vi "AO Python Interface.vi"(7 "Calling VI Ref":refnum<vi>) -> ()   [LabVIEW 2016]
uses:
  AO Python Controls/AO Python Data Type.ctl
  AO Python Controls/AO Python Units.ctl
  AO Python Controls/AO Python Vector Type.ctl
  AO Python Controls/AO Python Update Type.ctl
  AO Python Controls/AO Python Notifier Element.ctl
  AO Python Controls/AO Python Actions.ctl
  Hardware Configuration/Hardware Configuration Controls/Device Type.ctl
  Hardware Configuration/Hardware Configuration Controls/Device Function.ctl
  AO Python Controls/AO Python System Configuration.ctl
  AO Python Controls/AO Python Command List Type.ctl
  AO Python Controls/AO Python Next Command Type.ctl
  AO Python Controls/AO Python Image Type.ctl
  AO Python Controls/AO Python Status Type.ctl
panel:
  out "Current Image":u16[][](graph)
  in  "Use ROI":bool
  out "Python Status":string
  out "Command List":string[](array[string])
  in  "Fake Image":bool
  out "Command from Python":string
  in  "AO Data":T1={"LVCommand"="run_sensorless", "vector"=[], "flat_on"=1, "units"=enum."rad", "vector_type"=enum."zernike", "update_type"=enum."absolute"}
  in  "Send Command":bool
  in  "Quit":bool
  # "run_sensorless\nupdate\nquery_commands"
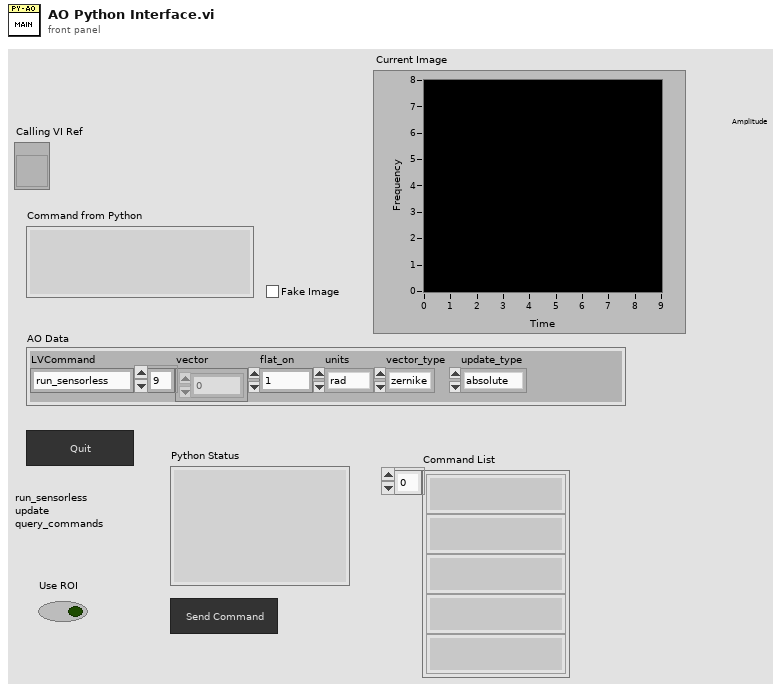
[diagram p1: front panel]
types:
  T1 = typedef "AO Python Data Type.ctl" = cluster{"LVCommand":string, "vector":dbl[], "flat_on":i32, "units":T2, "vector_type":T3, "update_type":T4}
  T2 = typedef "AO Python Units.ctl" = enum16{"rad", "nm"}
  T3 = typedef "AO Python Vector Type.ctl" = enum16{"zernike", "actuators", "zernike_highNA", "dm_modes1"}
  T4 = typedef "AO Python Update Type.ctl" = enum16{"absolute", "relative"}
  T5 = typedef "AO Python Actions.ctl" = enum16{"Error Check", "Open Connection", "Send Configuration", "Send Command", "Wait for Command", "Get Image", "Update DM", "Get Status", "Quit"}
  T6 = typedef "AO Python Notifier Element.ctl" = cluster{"Actions":T5, "Received?":bool, "Running?":bool, "AO Data":T1, "Command List":string[], "Python Status":string, "Error":errorcluster}
  T7 = typedef "Device Function.ctl" = enum16{"Primary", "Secondary", "Overview", "Wide Field Drift Correction", "642 nm Excitation", "560 nm Excitation", "546 nm Excitation", "488 nm Excitation", "405 nm Excitation", "Objective Drift Correction", "Objective XY", "Objective Z", "Sample XY", "Sample Coarse Z", "Sample Z", "4Pi Lower", "4Pi Upper", "Adj Cavity"}
  T8 = typedef "Device Type.ctl" = enum16{"AOTF", "Camera", "Deformable Mirror", "Laser", "Shutter", "Stage"}
  T9 = typedef "AO Python Command List Type.ctl" = cluster{"CommandList":string[]}
  T10 = typedef "AO Python System Configuration.ctl" = cluster{"stack_size":u16[], "fov":dbl[]}
  T11 = typedef "AO Python Next Command Type.ctl" = cluster{"NextCommand":string}
  T12 = typedef "AO Python Image Type.ctl" = cluster{"stack":dbl[][][]}
  T13 = typedef "AO Python Status Type.ctl" = cluster{"ack":string}
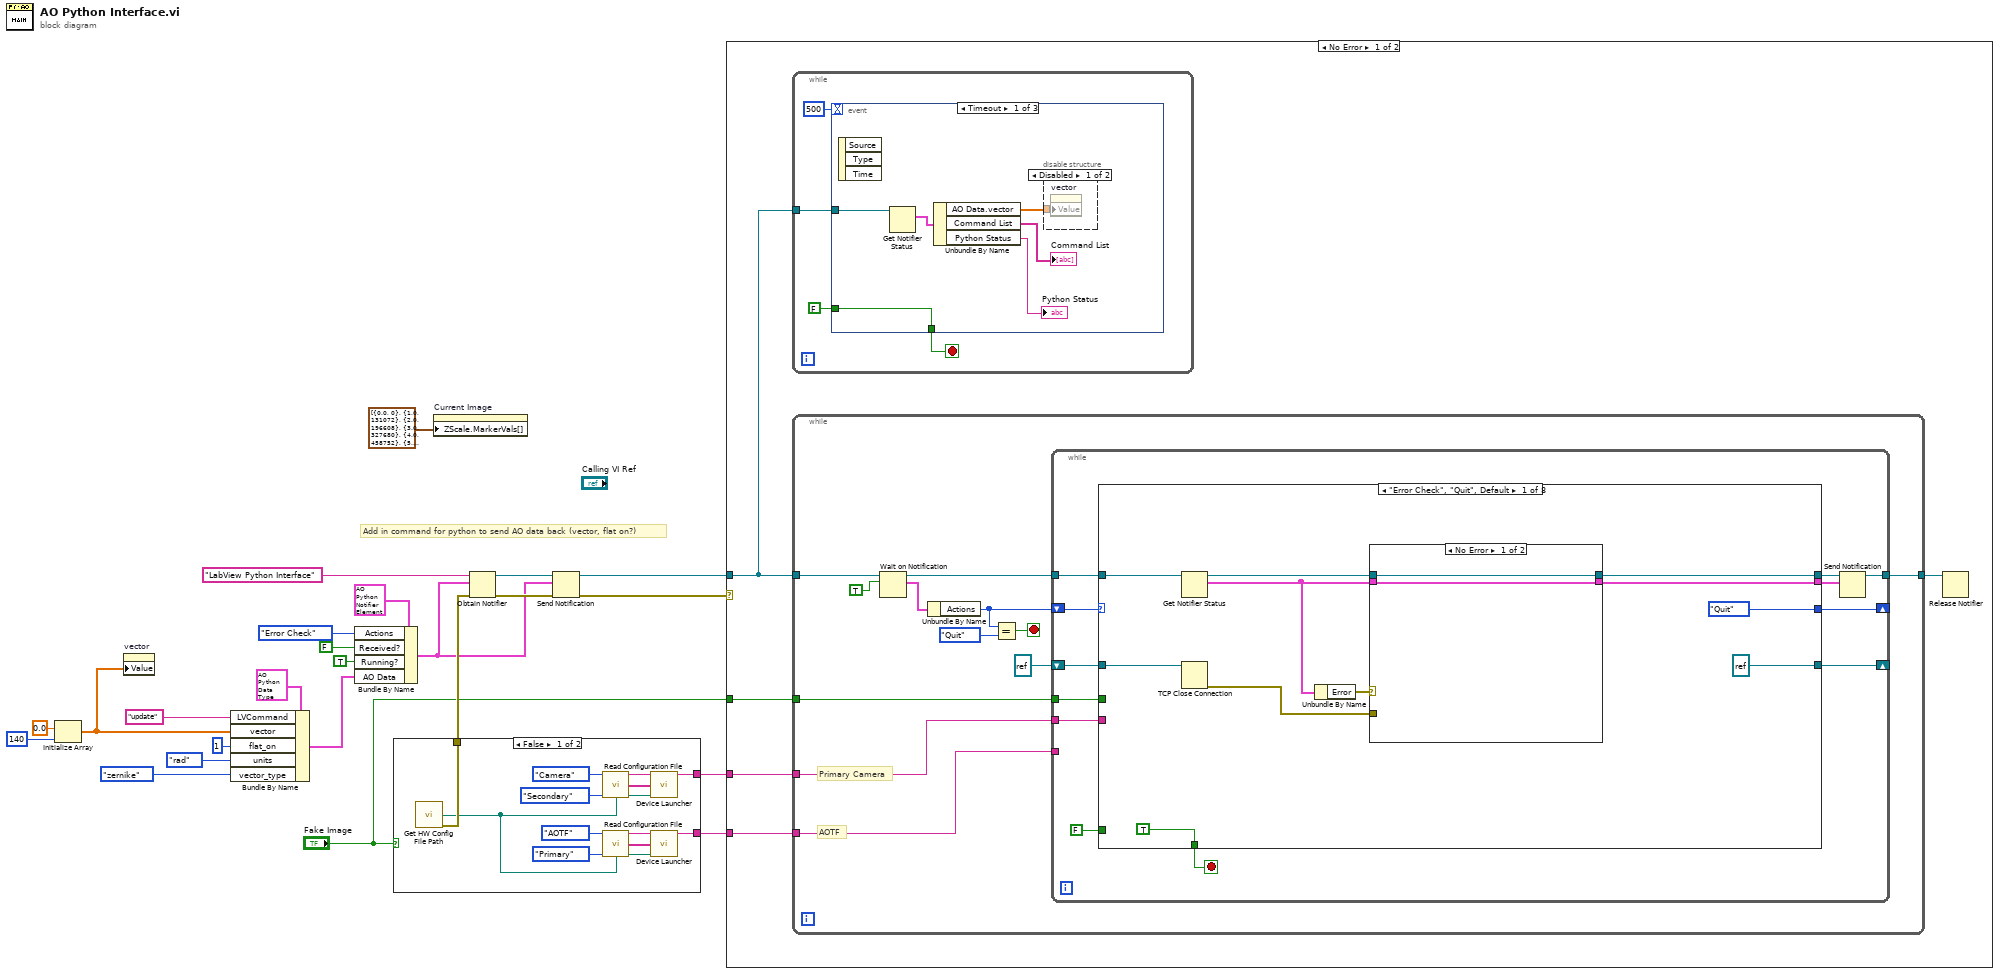
[diagram p0: block diagram]
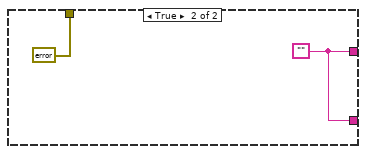
[diagram p2: hidden frame]
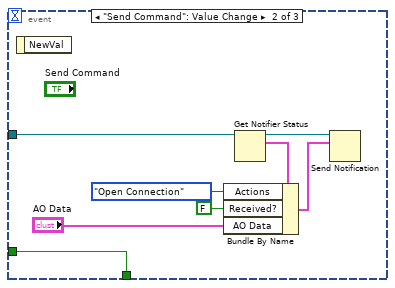
[diagram p4: hidden frame]
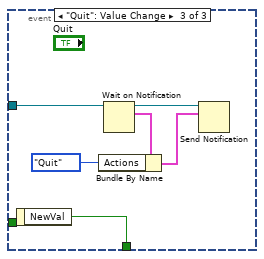
[diagram p5: hidden frame]
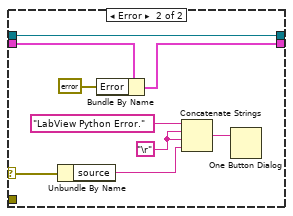
[diagram p6: hidden frame]
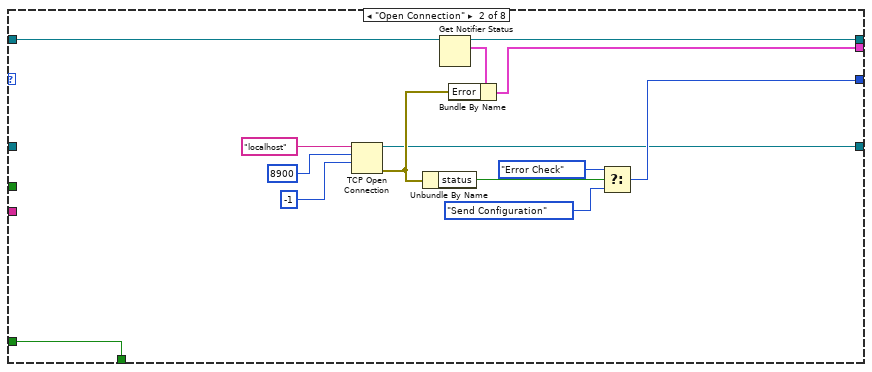
[diagram p7: hidden frame]
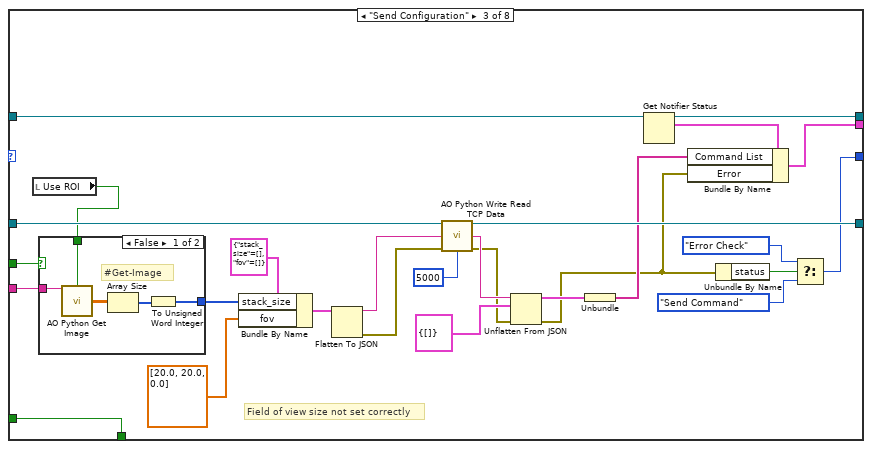
[diagram p8: hidden frame]
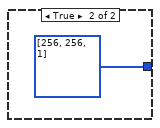
[diagram p9: hidden frame]
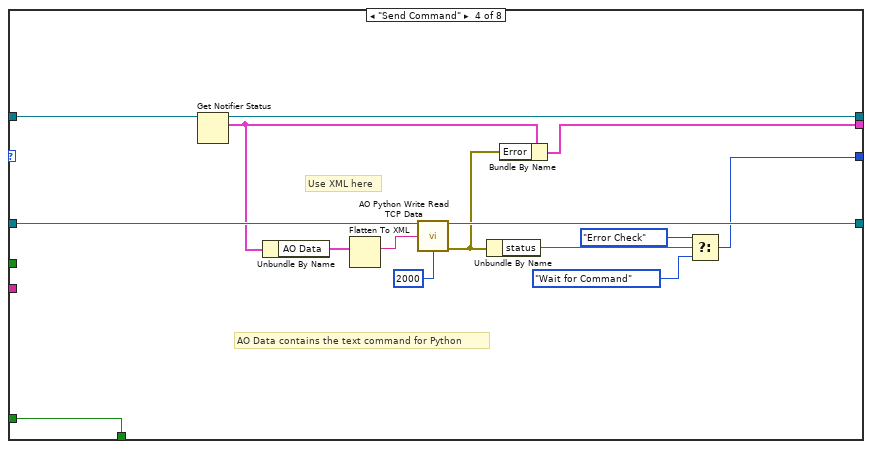
[diagram p10: hidden frame]
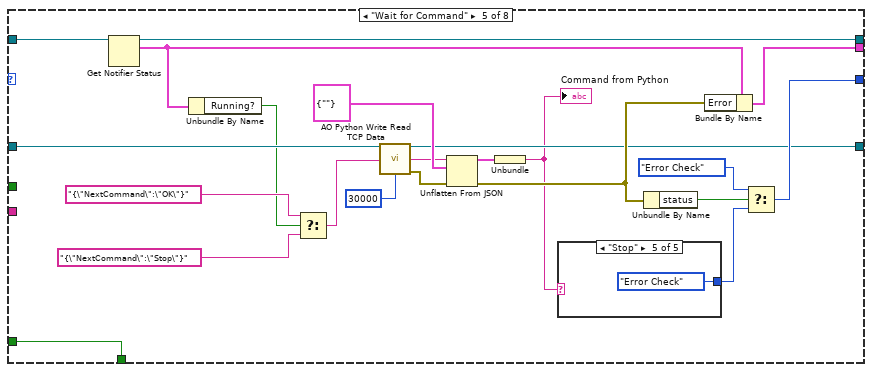
[diagram p11: hidden frame]
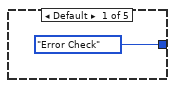
[diagram p12: hidden frame]
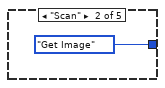
[diagram p13: hidden frame]
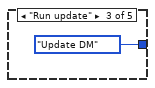
[diagram p14: hidden frame]
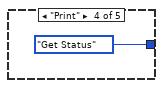
[diagram p15: hidden frame]
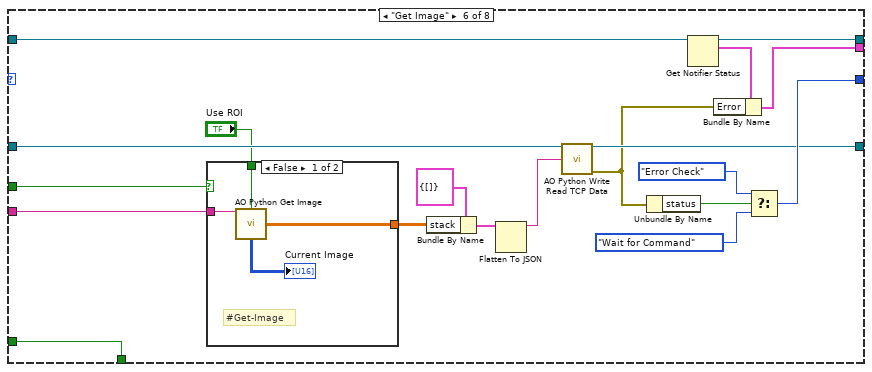
[diagram p16: hidden frame]
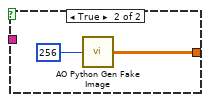
[diagram p17: hidden frame]
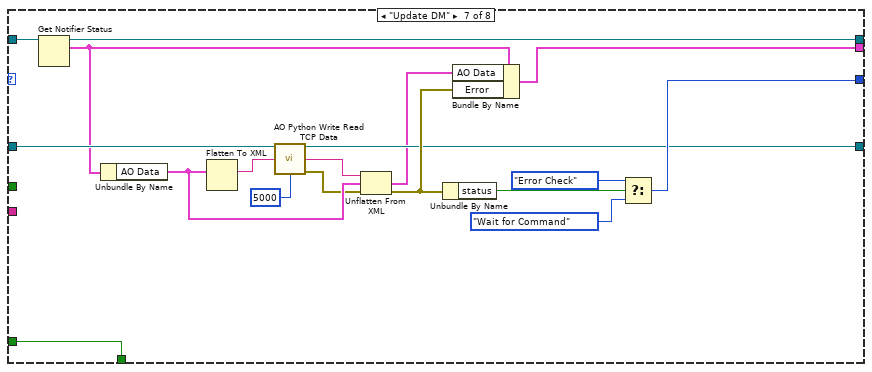
[diagram p18: hidden frame]
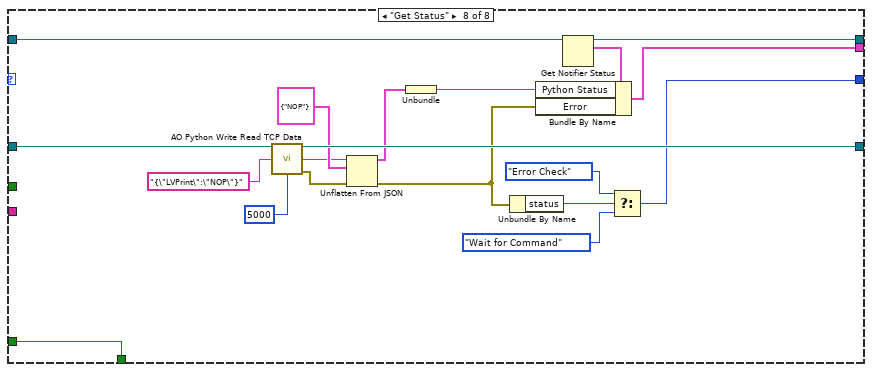
[diagram p19: hidden frame]
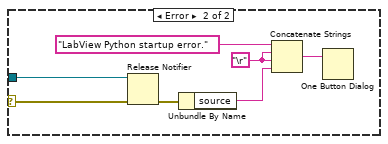
[diagram p20: hidden frame]
diagram:
  # "Add in command for python to send AO data back (vector, flat on?)"
  n1 = Initialize Array(0.0 ("element"), 140 ("dimension size")) -> (w1:dbl[])
  n2 = property on="vector" class="Arr (strict)"("Value"=w1) -> ()  [unwired: 2 in, 2 out]
  n3 = Bundle By Name(cluster=T1 {"LVCommand"="Default", "vector"=[], "flat_on"=1, "units"=enum."rad", "vector_type"=enum."zernike", "update_type"=enum."absolute"} ("input cluster"), "LVCommand"="update", "vector"=w1, "flat_on"=1 ("Flat On?"), "units"=AO_Python_Units."rad" ("Units"), "vector_type"=AO_Python_Vector_Type."zernike" ("Vector Type")) -> (w10:T1)
  n4 = Bundle By Name(cluster=T6 {"Actions"=enum."Send Command", "Received?"=FALSE, "Running?"=FALSE, "AO Data"={"LVCommand"="", "vector"=[], "flat_on"=1, "units"=enum."rad", "vector_type"=enum."zernike", "update_type"=enum."absolute"}, "Command List"=[], "Python Status"="", "Error"={"status"=FALSE, "code"=0, "source"=""}} ("LabView Python Notifier Element"), "Actions"=AO_Python_Actions."Error Check", "Received?"=FALSE, "Running?"=TRUE, "AO Data"=w10) -> (w4:T6)
  n5 = case shown="False" "Fake Image" {
    tunnel: [w38 w39] -> w23
    tunnel: [w37 errorcluster {"status"=FALSE, "code"=0, "source"=""} ("Error")] -> w22
    tunnel: [w35 w39] -> w21
    frame False {
      n6 = call "Get HW Config File Path.vi"() -> ("File Path"=w36:path, "Error"=w37:errorcluster)  [unwired: 14 in]
      n7 = call "Read Configuration File.vi"("Device Type"=Device_Type."Camera", "Device Function"=Device_Function."Secondary", "Config File Path"=w36) -> ("Unique Notifier Name"=w34:string, "Device Ports/IDs/Channels"=w33:string[], "Device Engine Path"=w32:path)  [unwired: 9 in, 1 out]
      n8 = call "Read Configuration File.vi"("Device Type"=Device_Type."AOTF", "Device Function"=Device_Function."Primary", "Config File Path"=w36) -> ("Unique Notifier Name"=w25:string, "Device Ports/IDs/Channels"=w26:string[], "Device Engine Path"=w27:path)  [unwired: 9 in, 1 out]
      n9 = call "Device Launcher.vi"("Notifier Name"=w34, "Device Ports/IDs/Channels"=w33, "Device Engine Path"=w32) -> ("Notifier Name"=w38:string)  [unwired: 11 in, 1 out]
      n10 = call "Device Launcher.vi"("Notifier Name"=w25, "Device Ports/IDs/Channels"=w26, "Device Engine Path"=w27) -> ("Notifier Name"=w35:string)  [unwired: 11 in, 1 out]
    }
    frame True {
      w39 = ""
    }
  }
  n11 = property on="Current Image" class="IntGraph (strict)"("ZScale.MarkerVals[]"=cluster{dbl, u32}[] [{0.0, 0}, {1.0, 131072}, {2.0, 196608}, {3.0, 327680}, {4.0, 458752}, {5.0, 589824}, {6.0, 720896}, {7.0, 851971}, {8.0, 983043}, {9.0, 1114115}, {10.0, 1245187}, {11.0, 1376259}, {12.0, 1507331}, {13.0, 1638403}, {14.0, 1769475}, {15.0, 1769479}, {16.0, 2031623}, {17.0, 2162695}, {18.0, 2293767}, {19.0, 2424839}, {20.0, 2555911}, {21.0, 2686983}, {22.0, 2818055}, {23.0, 2949127}, {24.0, 3080203}, {25.0, 3211275}, {26.0, 3342347}, {27.0, 3473419}, {28.0, 3604491}, {29.0, 3735563}, {30.0, 3866635}, {31.0, 3867403}, {32.0, 4129547}, {33.0, 4260619}, {34.0, 4391691}, {35.0, 4522763}, {36.0, 4653839}, {37.0, 4784911}, {38.0, 4915983}, {39.0, 5178127}, {40.0, 5309199}, {41.0, 5440271}, {42.0, 5571343}, {43.0, 5702415}, {44.0, 5703439}, {45.0, 5965583}, {46.0, 6096655}, {47.0, 6227727}, {48.0, 6358799}, {49.0, 6489871}, {50.0, 6620943}, {51.0, 6752015}, {52.0, 6883087}, {53.0, 7015183}, {54.0, 7146255}, {55.0, 7277327}, {56.0, 7408399}, {57.0, 7539471}, {58.0, 7670543}, {59.0, 7801615}, {60.0, 8063759}, {61.0, 8194831}, {62.0, 8326927}, {63.0, 8457999}, {64.0, 8589075}, {65.0, 8720147}, {66.0, 8851219}, {67.0, 8982291}, {68.0, 9113363}, {69.0, 9114387}, {70.0, 9376531}, {71.0, 9507603}, {72.0, 9638675}, {73.0, 9769747}, {74.0, 9901843}, {75.0, 10032915}, {76.0, 10163987}, {77.0, 10229523}, {78.0, 10295059}, {79.0, 10427155}, {80.0, 10558227}, {81.0, 10689299}, {82.0, 10820371}, {83.0, 10886931}, {84.0, 10952467}, {85.0, 11083539}, {86.0, 11214611}, {87.0, 11215635}, {88.0, 11477779}, {89.0, 11543315}, {90.0, 11608851}, {91.0, 11740947}, {92.0, 11806483}, {93.0, 11872019}, {94.0, 12004115}, {95.0, 12135187}, {96.0, 12266259}, {97.0, 12267283}, {98.0, 12398355}, {99.0, 12529427}, {100.0, 12530451}, {101.0, 12595987}, {102.0, 12530451}, {103.0, 12793619}, {104.0, 12794131}, {105.0, 12794643}, {106.0, 13056787}, {107.0, 13057299}, {108.0, 13057811}, {109.0, 13188883}, {110.0, 13320979}, {111.0, 13386515}, {112.0, 13452563}, {113.0, 13584147}, {114.0, 13584659}, {115.0, 13585171}, {116.0, 13585683}, {117.0, 13717267}, {118.0, 13848339}, {119.0, 13849363}, {120.0, 13849875}, {121.0, 13850387}, {122.0, 13981459}, {123.0, 14113555}, {124.0, 14114067}, {125.0, 14114579}, {126.0, 14115091}, {127.0, 14246675}, {128.0, 14377747}, {129.0, 14378771}, {130.0, 14379283}, {131.0, 14379539}, {132.0, 14379795}, {133.0, 14380819}, {134.0, 14511891}, {135.0, 14643987}, {136.0, 14644503}, {137.0, 14645015}, {138.0, 14645527}, {139.0, 14646039}, {140.0, 14646551}, {141.0, 14778135}, {142.0, 14909207}, {143.0, 14910231}, {144.0, 14910747}, {145.0, 14911259}, {146.0, 14911771}, {147.0, 14912283}, {148.0, 14912797}, {149.0, 15044383}, {150.0, 15175455}, {151.0, 15175967}, {152.0, 15176479}, {153.0, 15176991}, {154.0, 15177507}, {155.0, 15178019}, {156.0, 15178531}, {157.0, 15310115}, {158.0, 15441701}, {159.0, 15441959}, {160.0, 15442215}, {161.0, 15442727}, {162.0, 15443243}, {163.0, 15443755}, {164.0, 15444269}, {165.0, 15444783}, {166.0, 15444783}, {167.0, 15576367}, {168.0, 15707953}, {169.0, 15708467}, {170.0, 15708979}, {171.0, 15708981}, {172.0, 15708983}, {173.0, 15710011}, {174.0, 15710523}, {175.0, 15711037}, {176.0, 15711039}, {177.0, 15711553}, {178.0, 15843139}, {179.0, 15974213}, {180.0, 15974215}, {181.0, 15974217}, {182.0, 15974219}, {183.0, 15975755}, {184.0, 15976271}, {185.0, 15976785}, {186.0, 15977299}, {187.0, 15977301}, {188.0, 15977815}, {189.0, 15978327}, {190.0, 15978331}, {191.0, 16109917}, {192.0, 16241503}, {193.0, 16241505}, {194.0, 16242019}, {195.0, 16242535}, {196.0, 16242537}, {197.0, 16242539}, {198.0, 16243563}, {199.0, 16243567}, {200.0, 16244081}, {201.0, 16244595}, {202.0, 16244599}, {203.0, 16244601}, {204.0, 16244603}, {205.0, 16245627}, {206.0, 16245631}, {207.0, 16245633}, {208.0, 16246147}, {209.0, 16246663}, {210.0, 16377735}, {211.0, 16508811}, {212.0, 16508815}, {213.0, 16509839}, {214.0, 16509843}, {215.0, 16509845}, {216.0, 16509847}, {217.0, 16510361}, {218.0, 16510875}, {219.0, 16510879}, {220.0, 16510881}, {221.0, 16510883}, {222.0, 16511399}, {223.0, 16511911}, {224.0, 16511915}, {225.0, 16511917}, {226.0, 16511919}, {227.0, 16511923}, {228.0, 16512437}, {229.0, 16512951}, {230.0, 16512955}, {231.0, 16512957}, {232.0, 16512959}, {233.0, 16512961}, {234.0, 16512963}, {235.0, 16512967}, {236.0, 16513481}, {237.0, 16513995}, {238.0, 16513999}, {239.0, 16514001}, {240.0, 16514003}, {241.0, 16514005}, {242.0, 16514007}, {243.0, 16514011}, {244.0, 16514013}, {245.0, 16514015}, {246.0, 16514019}, {247.0, 16514021}, {248.0, 16514023}, {249.0, 16514027}, {250.0, 16514029}, {251.0, 16514031}, {252.0, 16514035}, {253.0, 16514037}, {254.0, 16514039}, {255.0, 16514043}] ("Z Scale.Marker Values[]")) -> ()  [unwired: 2 in, 2 out]
  n12 = Obtain Notifier(name (unnamed)="LabView Python Interface", notification data type=w4, error in (no error)=w22) -> (notifier out=w8:refnum<notifier>, error out=w7:errorcluster)  [unwired: 1 in, 1 out]
  n13 = Send Notification(notification=w4, notifier=w8, error in (no error)=w7) -> (notifier out=w6:refnum<notifier>, error out=w5:errorcluster)
  n14 = case shown="No Error" w5 {
    selector: w5 -> [_ w268]
    tunnel: w6 -> [w42 w274]
    tunnel: w23 -> [w45 _]
    tunnel: w21 -> [w43 _]
    tunnel: "Fake Image" -> [w41 _]
    frame No Error {
      n15 = while {
        tunnel: w42 -> [w47]
        stop <- w49 stop-if-true
        n16 = event shown="[0] Timeout" {
          selector: _ -> [_ _ _]
          dyn-events: _ -> [_ _ _]
          timeout: 500 -> [_ _ _]
          tunnel: [w55 w64 w70] -> w49
          tunnel: FALSE -> [w55 w64 _]
          tunnel: w47 -> [w54 w59 w69]
          event Timeout {
            n17 = event-data() -> ()  [unwired: 1 in, 3 out]
            n18 = Get Notifier Status(notifier=w54) -> (current notification=w53:T6)  [unwired: 1 in, 4 out]
            n19 = Unbundle By Name(w53) -> ("AO Data.vector"=w52:dbl[], "Command List"=→"Command List":string[], "Python Status"=→"Python Status":string)
            n20 = disable-structure shown="Disabled" {
              disable-tunnel: w52 -> [w56 _]
              frame Disabled {
                n21 = property on="vector" class="Arr (strict)"("Value"=w56) -> ()  [unwired: 2 in, 2 out]
              }
              frame Enabled {
              }
            }
          }
          event "Send Command": Value Change {
            n22 = event-data() -> ()  [unwired: 1 in, 1 out]
            n23 = Get Notifier Status(notifier=w59) -> (notifier out=w63:refnum<notifier>, current notification=w62:T6)  [unwired: 1 in, 3 out]
            n24 = Bundle By Name(cluster=w62, "Actions"=AO_Python_Actions."Open Connection", "Received?"=FALSE, "AO Data"="AO Data") -> (w60:T6)
            n25 = Send Notification(notification=w60, notifier=w63) -> ()  [unwired: 1 in, 2 out]
          }
          event "Quit": Value Change {
            n26 = event-data() -> ("NewVal"=w70:bool)  [unwired: 1 in]
            n27 = Wait on Notification(notifier=w69) -> (notifier out=w68:refnum<notifier>, notification=w67:T6)  [unwired: 3 in, 2 out]
            n28 = Bundle By Name(cluster=w67, "Actions"=AO_Python_Actions."Quit") -> (w65:T6)
            n29 = Send Notification(notification=w65, notifier=w68) -> ()  [unwired: 1 in, 2 out]
          }
        }
      }
      n30 = while {
        tunnel: w42 -> [w82]
        tunnel: w45 -> [w76]
        tunnel: [w75] -> w44
        tunnel: w43 -> [w74]
        tunnel: w41 -> [w71]
        stop <- w78 stop-if-true
        # "AOTF"
        # "Primary Camera"
        n31 = Wait on Notification(notifier=w82, ignore previous (F)=TRUE) -> (notifier out=w80:refnum<notifier>, notification=w77:T6)  [unwired: 2 in, 2 out]
        n32 = Unbundle By Name(w77) -> ("Actions"=w79:T5)
        n33 = Equal?(x=w79, y=AO_Python_Actions."Quit") -> (x = y?=w78:bool)
        n34 = while {
          tunnel: w80 -> [w93]
          shift-right: [w92] -> _
          shift-left: w79 -> [w94]
          tunnel: w76 -> [w84]
          tunnel: [w86] -> w75
          tunnel: w74 -> [_]
          shift-right: [w88] -> _
          shift-left: refnum<k5> refnum ("connection ID") -> [w90]
          tunnel: w71 -> [w83]
          stop <- w91 stop-if-true
          n35 = case shown="\"Error Check\", \"Quit\", Default" w94 {
            tunnel: w93 -> [w97 w119 w137 w166 w181 w211 w234 w251]
            tunnel: [AO_Python_Actions."Quit" ("y") w122 w151 w167 w192 w222 w241 w260] -> w92
            tunnel: [TRUE w127 w157 w178 w200 w224 w238 w267] -> w91
            tunnel: w90 -> [w99 _ w144 w177 w199 w218 w243 w266]
            tunnel: FALSE -> [_ w127 w157 w178 w200 w224 w238 w267]
            tunnel: [refnum<k5> refnum ("connection ID") w120 w156 w173 w185 w217 w237 w264] -> w88
            tunnel: [w104 w118 w136 w165 w180 w210 w233 w250] -> w87
            tunnel: [w103 w123 w155 w168 w191 w223 w242 w261] -> w85
            tunnel: w84 -> [_ _ w134 _ _ w208 _ _]
            tunnel: w83 -> [_ _ w132 _ _ w207 _ _]
            frame "Error Check", "Quit", Default {
              n36 = Get Notifier Status(notifier=w97) -> (notifier out=w96:refnum<notifier>, current notification=w95:T6)  [unwired: 1 in, 3 out]
              n37 = TCP Close Connection(connection ID=w99) -> (error out=w98:errorcluster)  [unwired: 2 in, 1 out]
              n38 = Unbundle By Name(w95) -> ("Error"=w105:errorcluster)
              n39 = case shown="No Error" w105 {
                selector: w105 -> [_ w111]
                tunnel: w95 -> [w106 w115]
                tunnel: [w107 w113] -> w104
                tunnel: w96 -> [w107 w113]
                tunnel: [w106 w112] -> w103
                tunnel: w98 -> [_ _]
                frame No Error {
                }
                frame Error {
                  w109 = "\r"
                  n40 = Unbundle By Name(w111) -> ("source"=w108:string)
                  n41 = Bundle By Name(cluster=w115, "Error"=errorcluster {"status"=FALSE, "code"=0, "source"=""}) -> (w112:T6)
                  n42 = Concatenate Strings("LabView Python Error." ("string"), w109, w109, w108) -> (w116:string)
                  n43 = One Button Dialog(message=w116) -> ()  [unwired: 1 in, 1 out]
                }
              }
            }
            frame "Open Connection" {
              n44 = TCP Open Connection(address="localhost", remote port or service name=u16 8900, timeout ms (60000)=-1) -> (connection ID=w120:refnum<k5>, error out=w121:errorcluster)  [unwired: 2 in]
              n45 = Unbundle By Name(w121) -> ("status"=w126:bool)
              n46 = Get Notifier Status(notifier=w119) -> (notifier out=w118:refnum<notifier>, current notification=w117:T6)  [unwired: 1 in, 3 out]
              n47 = Bundle By Name(cluster=w117, "Error"=w121) -> (w123:T6)
              n48 = Select(t=AO_Python_Actions."Error Check", s=w126, f=AO_Python_Actions."Send Configuration" ("y")) -> (s? t:f=w122:T5)
            }
            frame "Send Configuration" {
              # "Field of view size not set correctly"
              n49 = local read "Use ROI"() -> (w131:bool)
              n50 = case shown="False" w132 {
                tunnel: w134 -> [w162 _]
                tunnel: [w159 u16[] [256, 256, 1] ("stack_size")] -> w133
                tunnel: w131 -> [w158 _]
                frame False {
                  # "#Get-Image"
                  n51 = call "AO Python Get Image.vi"("Camera Notifier"=w162, "Use ROI"=w158) -> ("Image Out"=w161:dbl[][][])  [unwired: 12 in, 1 out]
                  n52 = Array Size(array=w161) -> (size(s)=w160:i32[])
                  n53 = To Unsigned Word Integer(number=w160) -> (unsigned 16bit integer=w159:u16[])
                }
                frame True {
                }
              }
              n54 = Bundle By Name(cluster=T10 {"stack_size"=[], "fov"=[]} ("AO Python System Configuration"), "stack_size"=w133, "fov"=dbl[] [20.0, 20.0, 0.0]) -> (w148:T10)
              n55 = Flatten To JSON(anything=w148) -> (JSON string=w147:string, 11:w146:errorcluster)  [unwired: 2 in]
              n56 = call "AO Python Write Read TCP Data.vi"("Connection ID"=w144, "Write String"=w147, "Error"=w146, "Timeout (ms)"=5000) -> ("Connection ID (Dup)"=w156:refnum<k5>, "Read String"=w141:string, "Error Out"=w139:errorcluster)  [unwired: 9 in]
              n57 = Unflatten From JSON(JSON string=w141, type and defaults=T9 {"CommandList"=[]}, error in (no error)=w139) -> (value=w143:T9, error out=w138:errorcluster)  [unwired: 4 in]
              n58 = Unbundle(w143) -> ("CommandList"=w140:string[])
              n59 = Get Notifier Status(notifier=w137) -> (notifier out=w136:refnum<notifier>, current notification=w135:T6)  [unwired: 1 in, 3 out]
              n60 = Bundle By Name(cluster=w135, "Command List"=w140, "Error"=w138) -> (w155:T6)
              n61 = Unbundle By Name(w138) -> ("status"=w154:bool)
              n62 = Select(t=AO_Python_Actions."Error Check", s=w154, f=AO_Python_Actions."Send Command" ("y")) -> (s? t:f=w151:T5)
            }
            frame "Send Command" {
              # "Use XML here"
              # "AO Data contains the text command for Python"
              n63 = Get Notifier Status(notifier=w166) -> (notifier out=w165:refnum<notifier>, current notification=w164:T6)  [unwired: 1 in, 3 out]
              n64 = Unbundle By Name(w164) -> ("AO Data"=w175:T1)
              n65 = Flatten To XML(anything=w175) -> (xml string=w174:string)
              n66 = call "AO Python Write Read TCP Data.vi"("Connection ID"=w177, "Write String"=w174, "Timeout (ms)"=2000) -> ("Connection ID (Dup)"=w173:refnum<k5>, "Error Out"=w172:errorcluster)  [unwired: 10 in, 1 out]
              n67 = Unbundle By Name(w172) -> ("status"=w171:bool)
              n68 = Bundle By Name(cluster=w164, "Error"=w172) -> (w168:T6)
              n69 = Select(t=AO_Python_Actions."Error Check", s=w171, f=AO_Python_Actions."Wait for Command" ("y")) -> (s? t:f=w167:T5)
            }
            frame "Wait for Command" {
              n70 = Get Notifier Status(notifier=w181) -> (notifier out=w180:refnum<notifier>, current notification=w179:T6)  [unwired: 1 in, 3 out]
              n71 = Unbundle By Name(w179) -> ("Running?"=w190:bool)
              n72 = Select(t="{\"NextCommand\":\"OK\"}", s=w190, f="{\"NextCommand\":\"Stop\"}") -> (s? t:f=w195:string)
              n73 = call "AO Python Write Read TCP Data.vi"("Connection ID"=w199, "Write String"=w195, "Timeout (ms)"=30000) -> ("Connection ID (Dup)"=w185:refnum<k5>, "Read String"=w183:string, "Error Out"=w184:errorcluster)  [unwired: 10 in]
              n74 = Unflatten From JSON(JSON string=w183, type and defaults=T11 {"NextCommand"=""}, error in (no error)=w184) -> (value=w187:T11, error out=w189:errorcluster)  [unwired: 4 in]
              n75 = Unbundle(w187) -> ("NextCommand"=w182:string)
              "Command from Python" <- w182
              n76 = case shown="\"Stop\"" w182 {
                tunnel: [AO_Python_Actions."Error Check" ("y") AO_Python_Actions."Get Image" ("y") AO_Python_Actions."Update DM" ("y") AO_Python_Actions."Get Status" ("y") AO_Python_Actions."Error Check" ("y")] -> w186
                frame Default {
                }
                frame "Scan" {
                }
                frame "Run update" {
                }
                frame "Print" {
                }
                frame "Stop" {
                }
              }
              n77 = Unbundle By Name(w189) -> ("status"=w194:bool)
              n78 = Bundle By Name(cluster=w179, "Error"=w189) -> (w191:T6)
              n79 = Select(t=AO_Python_Actions."Error Check" ("y"), s=w194, f=w186) -> (s? t:f=w192:T5)
            }
            frame "Get Image" {
              n80 = case shown="False" w207 {
                tunnel: [w227 w230] -> w214
                tunnel: w208 -> [w228 _]
                tunnel: "Use ROI" -> [w226 _]
                frame False {
                  # "#Get-Image"
                  n81 = call "AO Python Get Image.vi"("Camera Notifier"=w228, "Use ROI"=w226) -> ("Image Out"=w227:dbl[][][], "2D Image"=→"Current Image":u16[][])  [unwired: 12 in]
                }
                frame True {
                  n82 = call "AO Python Gen Fake Image.vi"("Size (pixels)"=256) -> ("Fake Image"=w230:dbl[][][])  [unwired: 14 in]
                }
              }
              n83 = Bundle By Name(cluster=T12 {"stack"=[]} ("Image Type"), "stack"=w214) -> (w213:T12)
              n84 = Flatten To JSON(anything=w213) -> (JSON string=w212:string)  [unwired: 2 in, 1 out]
              n85 = call "AO Python Write Read TCP Data.vi"("Connection ID"=w218, "Write String"=w212) -> ("Connection ID (Dup)"=w217:refnum<k5>, "Error Out"=w216:errorcluster)  [unwired: 11 in, 1 out]
              n86 = Unbundle By Name(w216) -> ("status"=w221:bool)
              n87 = Get Notifier Status(notifier=w211) -> (notifier out=w210:refnum<notifier>, current notification=w209:T6)  [unwired: 1 in, 3 out]
              n88 = Bundle By Name(cluster=w209, "Error"=w216) -> (w223:T6)
              n89 = Select(t=AO_Python_Actions."Error Check" ("y"), s=w221, f=AO_Python_Actions."Wait for Command" ("y")) -> (s? t:f=w222:T5)
            }
            frame "Update DM" {
              n90 = Get Notifier Status(notifier=w234) -> (notifier out=w233:refnum<notifier>, current notification=w232:T6)  [unwired: 1 in, 3 out]
              n91 = Unbundle By Name(w232) -> ("AO Data"=w239:T1)
              n92 = Flatten To XML(anything=w239) -> (xml string=w247:string)
              n93 = call "AO Python Write Read TCP Data.vi"("Connection ID"=w243, "Write String"=w247, "Timeout (ms)"=5000) -> ("Connection ID (Dup)"=w237:refnum<k5>, "Read String"=w236:string, "Error Out"=w235:errorcluster)  [unwired: 10 in]
              n94 = Unflatten From XML(xml string=w236, type=w239, error in (no error)=w235) -> (value=w231:T1, error out=w240:errorcluster)
              n95 = Unbundle By Name(w240) -> ("status"=w246:bool)
              n96 = Bundle By Name(cluster=w232, "AO Data"=w231, "Error"=w240) -> (w242:T6)
              n97 = Select(t=AO_Python_Actions."Error Check", s=w246, f=AO_Python_Actions."Wait for Command" ("y")) -> (s? t:f=w241:T5)
            }
            frame "Get Status" {
              n98 = call "AO Python Write Read TCP Data.vi"("Connection ID"=w266, "Write String"="{\"LVPrint\":\"NOP\"}", "Timeout (ms)"=5000) -> ("Connection ID (Dup)"=w264:refnum<k5>, "Read String"=w256:string, "Error Out"=w255:errorcluster)  [unwired: 10 in]
              n99 = Unflatten From JSON(JSON string=w256, type and defaults=T13 {"ack"="NOP"}, error in (no error)=w255) -> (value=w253:T13, error out=w254:errorcluster)  [unwired: 4 in]
              n100 = Unbundle(w253) -> ("ack"=w252:string)
              n101 = Unbundle By Name(w254) -> ("status"=w263:bool)
              n102 = Get Notifier Status(notifier=w251) -> (notifier out=w250:refnum<notifier>, current notification=w249:T6)  [unwired: 1 in, 3 out]
              n103 = Bundle By Name(cluster=w249, "Python Status"=w252, "Error"=w254) -> (w261:T6)
              n104 = Select(t=AO_Python_Actions."Error Check" ("y"), s=w263, f=AO_Python_Actions."Wait for Command" ("y")) -> (s? t:f=w260:T5)
            }
          }
          n105 = Send Notification(notification=w85, notifier=w87) -> (notifier out=w86:refnum<notifier>)  [unwired: 1 in, 1 out]
        }
      }
      n106 = Release Notifier(notifier=w44) -> ()  [unwired: 2 in, 3 out]
    }
    frame Error {
      w272 = "\r"
      n107 = Release Notifier(notifier=w274, error in (no error)=w268) -> (error out=w271:errorcluster)  [unwired: 1 in, 2 out]
      n108 = Unbundle By Name(w271) -> ("source"=w270:string)
      n109 = Concatenate Strings("LabView Python startup error.", w272, w272, w270) -> (w269:string)
      n110 = One Button Dialog(message=w269) -> ()  [unwired: 1 in, 1 out]
    }
  }
